vi "Parse State from Frame Name.vi"(6 "Wrap in Quotes? (FALSE)":bool, 7 "Category (Optional)":string, 11 "Frame or State Name":string) -> (0 "Has Category?":bool, 1 "is a Category Frame?":bool, 2 "State Name":string, 3 "Category Name":string, 4 "\"Category: State\" String":string, 5 "Idle Frame?":bool)   [LabVIEW 2020, in "JKI State Machine API.lvlib" / "JKI SM.lvclass"]
uses:
  JKI SM.lvclass
  <userlib>/_OpenG.lib/string/string.llb/Trim Whitespace (String)__ogtk.vi
  <userlib>/_OpenG.lib/string/string.llb/openg_string.lvlib
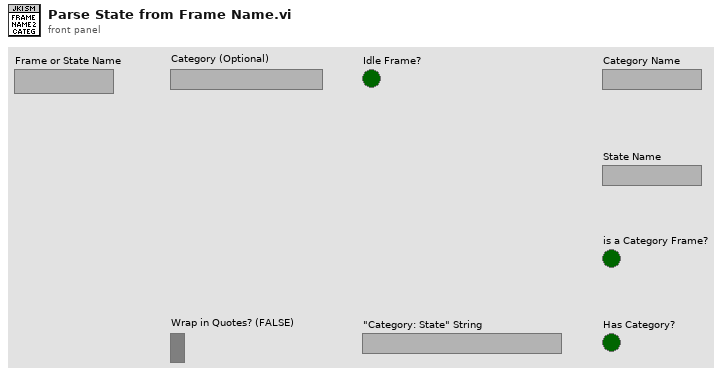
[diagram p1: front panel]
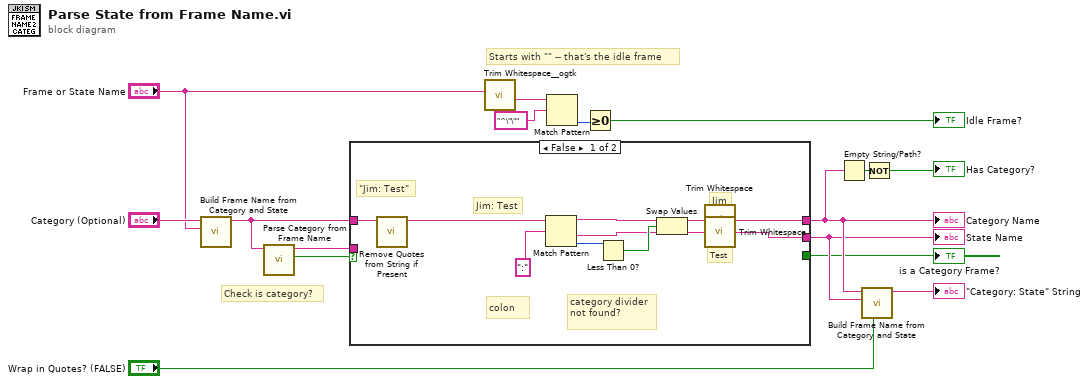
[diagram p0: block diagram]
diagram:
  # "Starts with \"\" -- that's the idle frame"
  # "Check is category?"
  n1 = call "Build Frame Name from Category and State.vi"("State Name"="Frame or State Name", "Category"="Category (Optional)") -> ("Frame Name"=w6:string)  [unwired: 9 in]
  n2 = call "Parse Category from Frame Name.vi"("Frame Name"=w6) -> ("is a Category?"=w10:bool, "Category Name"=w8:string)  [unwired: 9 in]
  n3 = case shown="False" w10 {
    selector: w10 -> [_ w29]
    tunnel: [_ w29] -> w11
    tunnel: [w23 w28] -> w15
    tunnel: w8 -> [_ w28]
    tunnel: w6 -> [w26 _]
    tunnel: [w24 _] -> w14
    frame False {
      # "category divider not found?"
      # "Test"
      # "Jim"
      # "Jim: Test"
      # "\"Jim: Test\""
      # "colon"
      n4 = call "Remove Quotes from String if Present.vi"("String"=w26) -> ("String with Quotes Removed"=w25:string)  [unwired: 10 in]
      n5 = Match Pattern(string=w25, regular expression=":") -> (before substring=w20:string, after substring=w18:string, offset past match=w22:i32)  [unwired: 1 in, 1 out]
      n6 = Less Than 0?(x=w22) -> (x < 0?=w21:bool)
      n7 = Swap Values(12:w20, 13:w21, 14:w18) -> (1:w19:string, 3:w17:string)
      n8 = call <vilib>:"Trim Whitespace.vi"("string"=w19) -> ("trimmed string"=w23:string)  [unwired: 1 in]
      n9 = call <vilib>:"Trim Whitespace.vi"("string"=w17) -> ("trimmed string"=w24:string)  [unwired: 1 in]
    }
    frame True {
    }
  }
  "is a Category Frame?" <- w11
  "Category Name" <- w15
  "State Name" <- w14
  n10 = call-poly <userlib>:"Trim Whitespace__ogtk.vi"("String in"="Frame or State Name") -> ("String out"=w4:string)  [unwired: 6 in]
  n11 = Match Pattern(string=w4, regular expression="^\"\"") -> (offset past match=w2:i32)  [unwired: 1 in, 3 out]
  n12 = Greater Or Equal To 0?(x=w2) -> (x >= 0?=→"Idle Frame?":bool)
  n13 = Empty String/Path?(string/path=w15) -> (empty?=w9:bool)
  n14 = call "Build Frame Name from Category and State.vi"("Wrap in Quotes? (TRUE)"="Wrap in Quotes? (FALSE)", "State Name"=w14, "Category"=w15) -> ("Frame Name"=→"\"Category: State\" String":string)  [unwired: 8 in]
  n15 = Not(x=w9) -> (.not. x?=→"Has Category?":bool)
